vi "ZM-ROOT-createResources.vi"(8 "error in (no error)":errorcluster, 11 "ZM-ROOT-root in":refnum<class "ZM-ROOT-root.lvclass">) -> (0 "error out":errorcluster, 3 "ZM-ROOT-root out":refnum<class "ZM-ROOT-root.lvclass">)   [LabVIEW 2020, in "ZM-ROOT-root.lvlib" / "ZM-ROOT-root.lvclass"]
doc: "Creates the root's resources in Pre Launch Init: the stop and error user events (ZM-ROOT-createEvents). If that fails, it destroys what was created (ZM-ROOT-close) and returns the original error, so the launch fails."
uses:
  ZM-ROOT-root.lvclass
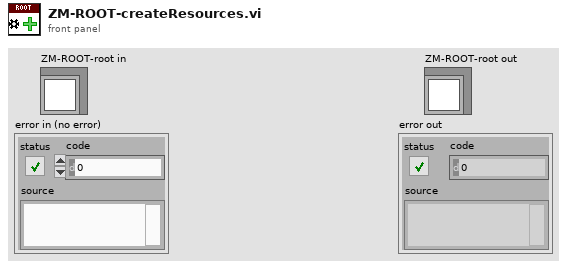
[diagram p1: front panel]
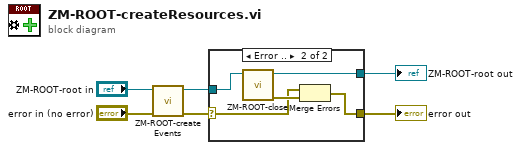
[diagram p0: block diagram]
diagram:
  n1 = call "ZM-ROOT-createEvents.vi"("error in (no error)"="error in (no error)", "ZM-ROOT-root in"="ZM-ROOT-root in") -> ("error out"=w3:errorcluster, "ZM-ROOT-root out"=w4:refnum<class "ZM-ROOT-root.lvclass">)  [unwired: 8 in]
  n2 = case shown="Error .." w3 {
    selector: w3 -> [w7 w9]
    tunnel: w4 -> [w8 w13]
    tunnel: [w8 w11] -> w2
    tunnel: [w7 w10] -> w1
    frame No Error {
    }
    frame Error {
      n3 = call "ZM-ROOT-close.vi"("ZM-ROOT-root in"=w13) -> ("error out"=w12:errorcluster, "ZM-ROOT-root out"=w11:refnum<class "ZM-ROOT-root.lvclass">)  [unwired: 9 in]
      n4 = Merge Errors(w9, w12) -> (w10:errorcluster)
    }
  }
  "ZM-ROOT-root out" <- w2
  "error out" <- w1
